vi "RT_Main.vi"(8 "error in (no error)":errorcluster={"status"=FALSE, "code"=0, "source"="\"\""}, 10 "controller configuration":string="CFG_SERVO", 11 "Hardware map":string="HW_MAP") -> (0 "error out":errorcluster={"status"=FALSE, "code"=0, "source"="\"\""}, 2 "status ok":bool, 3 "RT running status":string)   [LabVIEW 2026]
doc: "INTENT: Deterministic RT Controller Main coordinating hardware acquisition, servo position loop, and fault monitoring."
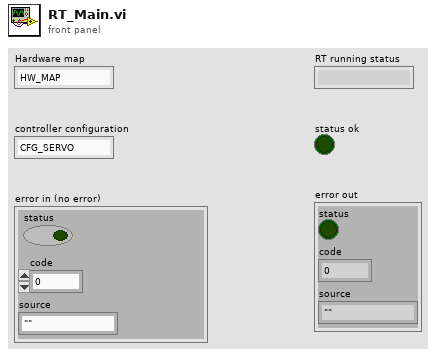
[diagram p1: front panel]
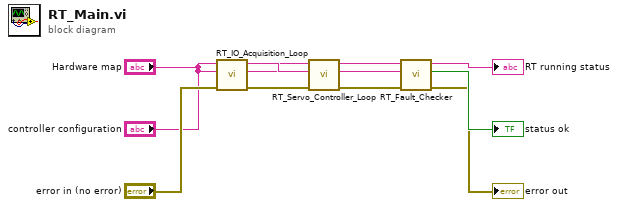
[diagram p0: block diagram]
diagram:
  n1 = call "RT_IO_Acquisition_Loop.vi"("error in (no error)"="error in (no error)", "sample policy"="controller configuration", "NI hardware references"="Hardware map") -> ("error out"=w5:errorcluster, "Typed process value updates"=w4:string)  [unwired: 6 in, 1 out]
  n2 = call "RT_Servo_Controller_Loop.vi"("error in (no error)"=w5, "encoder data"=w4, "Setpoint/mode"="controller configuration") -> ("error out"=w7:errorcluster, "Servo feedback/health"=w6:string)  [unwired: 6 in, 1 out]
  n3 = call "RT_Fault_Checker.vi"("error in (no error)"=w7, "watchdog status"="Hardware map", "Sensor/controller status"=w6) -> ("error out"=→"error out":errorcluster, "status ok"=→"status ok":bool, "FaultRecord and protective request"=→"RT running status":string)  [unwired: 6 in]
